vi "SMR_LabVIEW_V8.5.vi"() -> ()   [LabVIEW 2025]
uses:
  <vilib>/DAQmx/write.llb/DAQmx Write (Analog DBL 1Chan 1Samp).vi
  <vilib>/DAQmx/read.llb/DAQmx Read (Analog 1D DBL NChan 1Samp).vi
  <vilib>/DAQmx/read.llb/DAQmx Read (Analog 2D DBL NChan NSamp).vi
  <vilib>/Analysis/baseanly.llb/Mean (DBL).vi
  <vilib>/DAQmx/create/channels.llb/DAQmx Create Channel (AI-Temperature-Thermocouple).vi
  <vilib>/DAQmx/create/channels.llb/DAQmx Create Channel (AI-Voltage-Basic).vi
  <vilib>/DAQmx/create/channels.llb/DAQmx Create Channel (AO-Voltage-Basic).vi
  <vilib>/DAQmx/miscellaneous.llb/DAQmx Fill In Error Info.vi
  <vilib>/DAQmx/configure/timing.llb/DAQmx Timing (Sample Clock).vi
  <vilib>/addons/control/pid/pid.llb/PID (DBL).vi
  <vilib>/measure/maspectr.llb/FFT Power Spectrum and PSD for 1 Chan.vi
  <vilib>/measure/matone.llb/Extract Single Tone Information 1 Chan.vi
  <vilib>/addons/control/pid/NI_PID_pid.lvlib
  <vilib>/Analysis/NI_AALBase.lvlib
  <vilib>/ptbypt/NI_PtbyPt.lvlib
  <vilib>/measure/NI_MAPro.lvlib
panel:
  out "HW Valve Command (V)":dbl
  in  "HX Flow Setpoint (GPM)":dbl
  in  "Manual HW Valve Voltage (V)":dbl
  in  "HW Valve: Manual / PID":bool
  in  "PID gains for HW Valve":T1={"proportional gain (Kc)"=1.0, "integral time (Ti, min)"=0.01, "derivative time (Td, min)"=0.0} {"derivative time (Td, min)" format="%.3f"; "integral time (Ti, min)" format="%.3f"; "proportional gain (Kc)" format="%.3f"}
  out "Rod Power (W)":dbl
  out "Current Through Rod (A)":dbl
  out "Time in Steady State (s)":dbl
  in  "Steady-State Dwell (s)":dbl
  out "Main Loop Flow (GPM)":dbl
  out "FM Amplitude":dbl
  out "FM Frequency":dbl
  out "Spectrum":cluster{"f0":dbl, "df":dbl, "magnitude":dbl[]}(graph)
  out "Raw Signal":waveform(dbl)(graph)
  out "Smoothed HX Flow (GPM)":dbl
  out "Flow History":dbl(graph)
  out "HX Flow (GPM)":dbl
  out "Voltage Across Rod (V)":dbl format="%0.2f"
  out "Current Run Folder":path
  in  "Log Root Folder":path=path "C:/Users/LocalUser/Documents/GitHub/thermal-loop/resources/v0.1.1/data/001"
  out "Raw NI9201 \nVoltage Display":T2
  in  "Loop Period (ms)":dbl=1000.0
  in  "Stop":bool
  out "Auto Steady State Threshold (deg C/min)":dbl
  out "Max dT/dt (deg C/min)":dbl
  out "Temp Change Rate (deg C/min)":dbl
  out "5-Min Baseline Complete":bool
  out "Rate Window Ready":bool
  out "Steady State":bool
  in  "Voltage Limit (V)":dbl=10.0
  in  "Temperature Limit (C)":dbl=50.0
  in  "Pressure Limit (psi)":dbl=15.0
  out "Max Voltage":bool
  out "Max Temperature":bool
  out "Max Pressure":bool
  out "Heat Exchanger Pressure History":dbl(graph)
  out "Main Loop Pressure History":T3(graph)
  out "Overall Avg Pressure (psi)":dbl
  out "Heat Exchanger Pressure P6 (psi)":dbl
  out "Main Loop Avg Pressure (psi)":dbl
  out "Pressure Display":T4
  out "Overall Pressure History":T5(graph)
  out "Max Loop Pressure (psi)":dbl
  out "Heat Exchanger Temperature History":cluster{"Waveform":dbl, "Waveform":dbl}(graph)
  out "Main Loop Temeperature History":T6(graph)
  out "Heat Exchanger Avg Temp (deg C)":dbl
  out "Temperature Display":T7
  out "Overall Temperature History":T8(graph)
  out "Overall Avg Temp (deg C)":dbl
  out "Max Loop Temp (deg C)":dbl
  out "Final P-Valve Voltage (V)":dbl
  out "PID Trim Voltage (V)":dbl
  in  "PID Temp Setpoint (deg C)":dbl
  in  "Auto PID Enable":bool
  in  "Manual P-Valve Voltage (V)":dbl min=0.0 max=10.0
  out "Main Loop Avg Temp (deg C)":dbl
  # "HoneyWell Valve Control"
  # "Heat Exchanger Flow"
  # "Control/Troubleshoot"
  # "Steady State"
  # "Emergency Indicators"
  # "Pressure"
  # "Temperature"
  # "Proportional Valve Control"
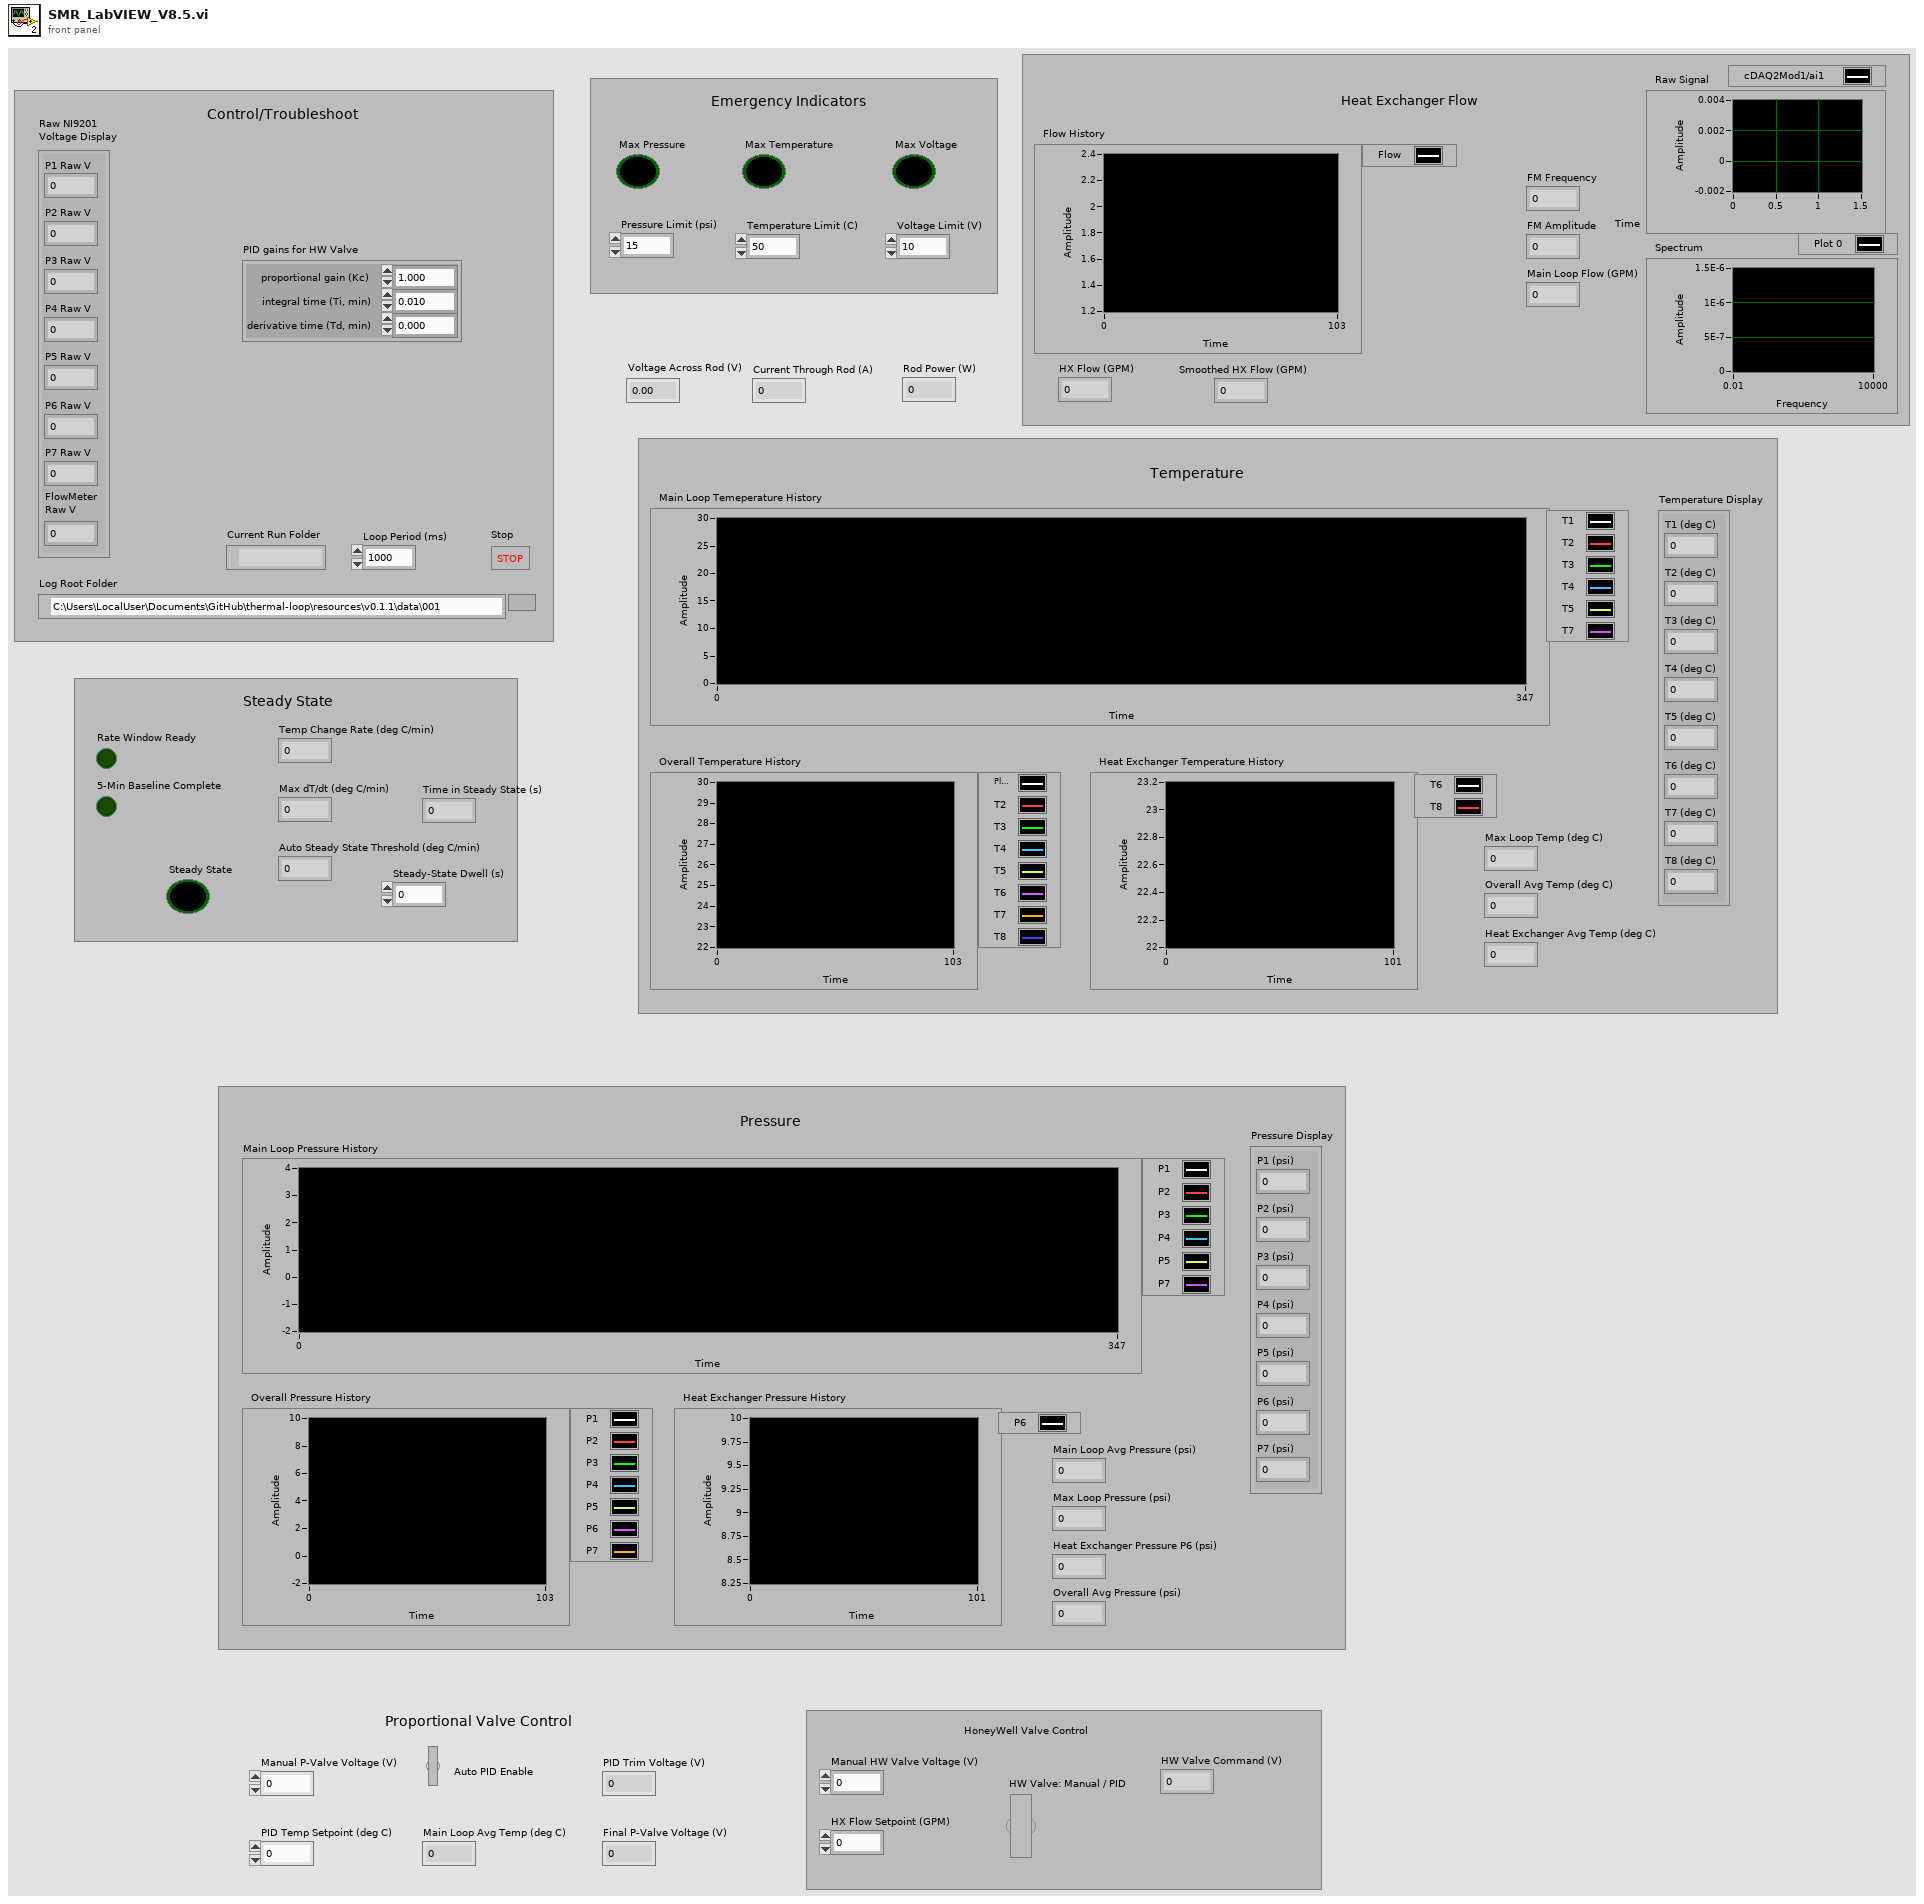
[diagram p1: front panel]
types:
  T1 = cluster{"proportional gain (Kc)":dbl, "integral time (Ti, min)":dbl, "derivative time (Td, min)":dbl}
  T2 = cluster{"P1 Raw V":dbl, "P2 Raw V":dbl, "P3 Raw V":dbl, "P4 Raw V":dbl, "P5 Raw V":dbl, "P6 Raw V":dbl, "P7 Raw V":dbl, "FlowMeter\nRaw V":dbl}
  T3 = cluster{"P1":dbl, "P2":dbl, "P3":dbl, "P4":dbl, "P5":dbl, "P7":dbl}
  T4 = cluster{"P1 (psi)":dbl, "P2 (psi)":dbl, "P3 (psi)":dbl, "P4 (psi)":dbl, "P5 (psi)":dbl, "P6 (psi)":dbl, "P7 (psi)":dbl}
  T5 = cluster{"P1":dbl, "P2":dbl, "P3":dbl, "P4":dbl, "P5":dbl, "P6":dbl, "P7":dbl}
  T6 = cluster{"Waveform":dbl, "Waveform":dbl, "Waveform":dbl, "Waveform":dbl, "Waveform":dbl, "Waveform":dbl}
  T7 = cluster{"T1 (deg C)":dbl, "T2 (deg C)":dbl, "T3 (deg C)":dbl, "T4 (deg C)":dbl, "T5 (deg C)":dbl, "T6 (deg C)":dbl, "T7 (deg C)":dbl, "T8 (deg C)":dbl}
  T8 = cluster{"Waveform":dbl, "Waveform":dbl, "Waveform":dbl, "Waveform":dbl, "Waveform":dbl, "Waveform":dbl, "Waveform":dbl, "Waveform":dbl}
  T9 = enum16{"open", "replace", "create", "open or create", "replace or create", "replace or create with confirmation"}
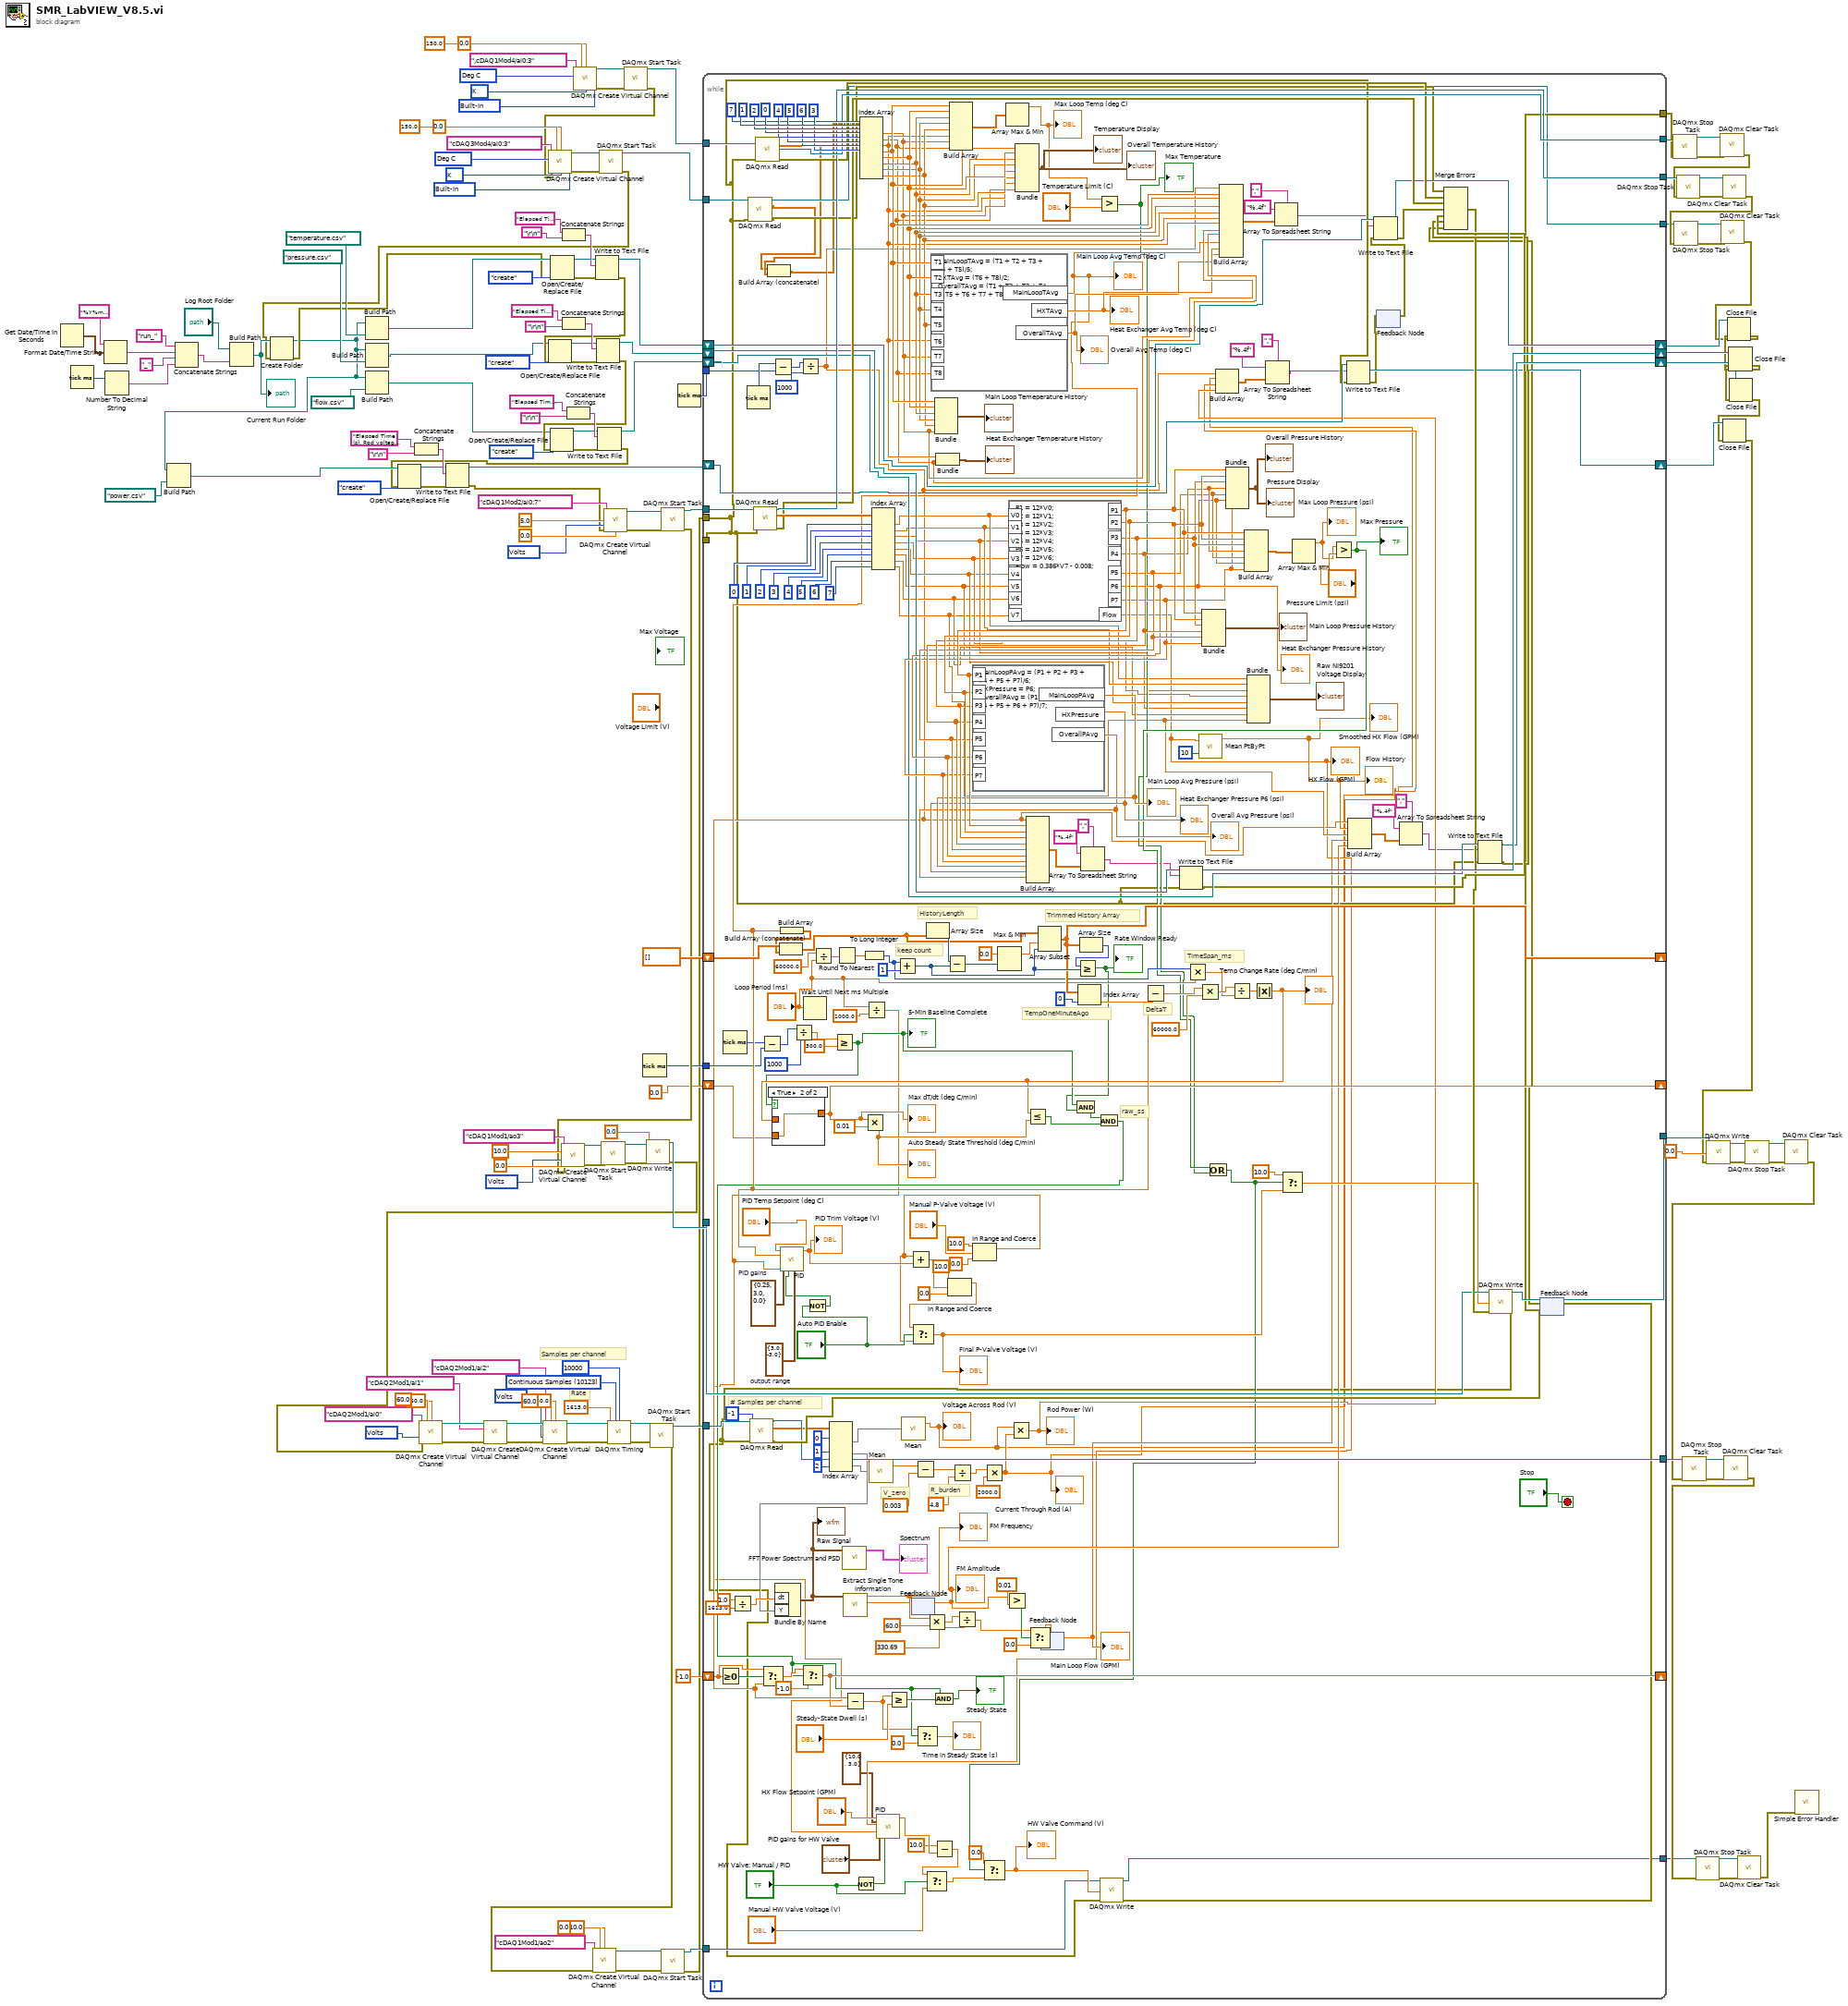
[diagram p0: block diagram]
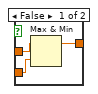
[diagram p2: hidden frame]
diagram:
  w17 = 10348 items=["Volts"=10348, "From Custom Scale"=10065] ("units")
  w34 = 10200 items=["Built-In"=10200, "Constant Value"=10116, "Channel"=10113] ("cjc source")
  w35 = 10073 items=["J"=10072, "K"=10073, "N"=10077, "R"=10082, "S"=10085, "T"=10086, "B"=10047, "E"=10055] ("thermocouple type")
  w36 = 10143 items=["Deg C"=10143, "Deg F"=10144, "Kelvins"=10325, "Deg R"=10145, "From Custom Scale"=10065] ("units")
  w66 = 10123 items=["Finite Samples"=10178, "Continuous Samples"=10123, "Hardware Timed Single Point"=12522] ("sample mode")
  w68 = 10348 items=["Volts"=10348, "From Custom Scale"=10065] ("units")
  w87 = 10348 items=["Volts"=10348, "From Custom Scale"=10065] ("units")
  w149 = 10200 items=["Built-In"=10200, "Constant Value"=10116, "Channel"=10113] ("cjc source")
  w150 = 10073 items=["J"=10072, "K"=10073, "N"=10077, "R"=10082, "S"=10085, "T"=10086, "B"=10047, "E"=10055] ("thermocouple type")
  w151 = 10143 items=["Deg C"=10143, "Deg F"=10144, "Kelvins"=10325, "Deg R"=10145, "From Custom Scale"=10065] ("units")
  w158 = 10348 items=["Volts"=10348, "From Custom Scale"=10065] ("units")
  # "Samples per channel"
  # "Rate"
  n1 = Get Date/Time In Seconds() -> (seconds since 1Jan1904=w108:timestamp)
  n2 = Tick Count (ms)() -> (millisecond timer value=w106:u32)
  n3 = Format Date/Time String(time format string (%c)="%Y%m%d_%H%M%S", seconds (now)=w108) -> (date/time string=w103:string)  [unwired: 1 in]
  n4 = Number To Decimal String(number=w106) -> (decimal integer string=w104:string)  [unwired: 1 in]
  n5 = Concatenate Strings("run_" ("string"), w103, "_" ("string"), w104) -> (w100:string)
  n6 = Build Path(base path="Log Root Folder", name or relative path=w100) -> (appended path=w99:path)
  "Current Run Folder" <- w99
  n7 = Concatenate Strings("Elapsed Time (s), Rod voltage (V), Rod Current (A), Rod Power (W)", "\r\n") -> (w53:string)
  n8 = Concatenate Strings("Elapsed Time (s),T1 (deg C),T2 (deg C),T3 (deg C),T4 (deg C),T5 (deg C),T6 (deg C),T7 (deg C),T8 (deg C),Main Loop Avg Temp (deg C),HX Avg Temp (deg C),Overall Avg Temp (deg C)", "\r\n") -> (w132:string)
  n9 = Concatenate Strings("Elapsed Time (s),P1 (psi),P2 (psi),P3 (psi),P4 (psi),P5 (psi),P6 (psi),P7 (psi),Main Loop Avg Pressure (psi),HX Pressure (psi),Overall Avg Pressure (psi)", "\r\n") -> (w130:string)
  n10 = Concatenate Strings("Elapsed Time (s),Heat Exchanger Flow (GPM),Flow Raw Voltage (V), Main Loop Flow (GPM), Flow Signal Amplitude (V)", "\r\n") -> (w126:string)
  n11 = call-poly <vilib>:"DAQmx Create Virtual Channel.vi"("maximum value"=150.0, "minimum value"=0.0, "physical channels"=tag ",cDAQ1Mod4/ai0:3", "cjc source"=w149, "units"=w151, "thermocouple type"=w150) -> ("task out"=w148:refnum<k21>, "error out"=w147:errorcluster)  [unwired: 8 in]
  n12 = call <vilib>:"DAQmx Start Task.vi"("task/channels in"=w148, "error in"=w147) -> ("task out"=w146:refnum<k21>, "error out"=w30:errorcluster)  [unwired: 12 in]
  n13 = call-poly <vilib>:"DAQmx Create Virtual Channel.vi"("maximum value"=150.0, "minimum value"=0.0, "physical channels"=tag "cDAQ3Mod4/ai0:3", "cjc source"=w34, "units"=w36, "error in"=w30, "thermocouple type"=w35) -> ("task out"=w33:refnum<k21>, "error out"=w32:errorcluster)  [unwired: 7 in]
  n14 = call <vilib>:"DAQmx Start Task.vi"("task/channels in"=w33, "error in"=w32) -> ("task out"=w28:refnum<k21>, "error out"=w29:errorcluster)  [unwired: 12 in]
  n15 = Create Folder(path (use dialog)=w99, error in=w29) -> (created path=w47:path, error out=w92:errorcluster)  [unwired: 1 in, 1 out]
  n16 = Build Path(base path=w47, name or relative path=path "power.csv") -> (appended path=w48:path)
  n17 = Build Path(base path=w47, name or relative path=path "temperature.csv") -> (appended path=w98:path)
  n18 = Build Path(base path=w47, name or relative path=path "pressure.csv") -> (appended path=w97:path)
  n19 = Build Path(base path=w47, name or relative path=path "flow.csv") -> (appended path=w96:path)
  n20 = Open/Create/Replace File(file path (use dialog)=w98, error in=w92, operation (0:open)=T9."create") -> (refnum out=w131:refnum<file>, error out=w115:errorcluster)  [unwired: 3 in, 1 out]
  n21 = Write to Text File(file (use dialog)=w131, text=w132, error in=w115) -> (refnum out=w122:refnum<file>, error out=w114:errorcluster)  [unwired: 1 in, 1 out]
  n22 = Open/Create/Replace File(file path (use dialog)=w97, error in=w114, operation (0:open)=T9."create") -> (refnum out=w129:refnum<file>, error out=w113:errorcluster)  [unwired: 3 in, 1 out]
  n23 = Write to Text File(file (use dialog)=w129, text=w130, error in=w113) -> (refnum out=w121:refnum<file>, error out=w112:errorcluster)  [unwired: 1 in, 1 out]
  n24 = Open/Create/Replace File(file path (use dialog)=w96, error in=w112, operation (0:open)=T9."create") -> (refnum out=w125:refnum<file>, error out=w111:errorcluster)  [unwired: 3 in, 1 out]
  n25 = Write to Text File(file (use dialog)=w125, text=w126, error in=w111) -> (refnum out=w120:refnum<file>, error out=w45:errorcluster)  [unwired: 1 in, 1 out]
  n26 = Open/Create/Replace File(file path (use dialog)=w48, error in=w45, operation (0:open)=T9."create") -> (refnum out=w52:refnum<file>, error out=w49:errorcluster)  [unwired: 3 in, 1 out]
  n27 = Write to Text File(file (use dialog)=w52, text=w53, error in=w49) -> (refnum out=w43:refnum<file>, error out=w44:errorcluster)  [unwired: 1 in, 1 out]
  n28 = call-poly <vilib>:"DAQmx Create Virtual Channel.vi"("maximum value"=5.0, "minimum value"=0.0, "physical channels"=tag "cDAQ1Mod2/ai0:7", "units"=w158, "error in"=w44) -> ("task out"=w157:refnum<k21>, "error out"=w156:errorcluster)  [unwired: 9 in]
  n29 = Tick Count (ms)() -> (millisecond timer value=w73:u32)
  n30 = call <vilib>:"DAQmx Start Task.vi"("task/channels in"=w157, "error in"=w156) -> ("task out"=w155:refnum<k21>, "error out"=w80:errorcluster)  [unwired: 12 in]
  n31 = call-poly <vilib>:"DAQmx Create Virtual Channel.vi"("maximum value"=10.0, "minimum value"=0.0, "physical channels"=tag "cDAQ1Mod1/ao3", "units"=w87, "error in"=w80) -> ("task out"=w86:refnum<k21>, "error out"=w85:errorcluster)  [unwired: 9 in]
  n32 = call <vilib>:"DAQmx Start Task.vi"("task/channels in"=w86, "error in"=w85) -> ("task out"=w84:refnum<k21>, "error out"=w83:errorcluster)  [unwired: 12 in]
  n33 = call-poly <vilib>:"DAQmx Write.vi"("task/channels in"=w84, "data"=0.0, "error in"=w83) -> ("task out"=w81:refnum<k21>, "error out"=w60:errorcluster)  [unwired: 10 in, 1 out]
  n34 = call-poly <vilib>:"DAQmx Create Virtual Channel.vi"("maximum value"=60.0, "minimum value"=-60.0, "physical channels"=tag "cDAQ2Mod1/ai0", "units"=w68, "error in"=w60) -> ("task out"=w57:refnum<k21>, "error out"=w56:errorcluster)  [unwired: 9 in]
  n35 = call-poly <vilib>:"DAQmx Create Virtual Channel.vi"("task in"=w57, "physical channels"=tag "cDAQ2Mod1/ai1", "error in"=w56) -> ("task out"=w21:refnum<k21>, "error out"=w19:errorcluster)  [unwired: 11 in]
  n36 = call-poly <vilib>:"DAQmx Create Virtual Channel.vi"("task in"=w21, "maximum value"=60.0, "minimum value"=-60.0, "physical channels"=tag "cDAQ2Mod1/ai2", "units"=w17, "error in"=w19) -> ("task out"=w20:refnum<k21>, "error out"=w18:errorcluster)  [unwired: 8 in]
  n37 = call-poly <vilib>:"DAQmx Timing.vi"("task/channels in"=w20, "sample mode"=w66, "samples per channel"=10000, "rate"=1613.0, "error in"=w18) -> ("task out"=w64:refnum<k21>, "error out"=w63:errorcluster)  [unwired: 9 in]
  n38 = call <vilib>:"DAQmx Start Task.vi"("task/channels in"=w64, "error in"=w63) -> ("task out"=w59:refnum<k21>, "error out"=w8:errorcluster)  [unwired: 12 in]
  n39 = call-poly <vilib>:"DAQmx Create Virtual Channel.vi"("maximum value"=10.0, "minimum value"=0.0, "physical channels"=tag "cDAQ1Mod1/ao2", "error in"=w8) -> ("task out"=w11:refnum<k21>, "error out"=w10:errorcluster)  [unwired: 10 in]
  n40 = call <vilib>:"DAQmx Start Task.vi"("task/channels in"=w11, "error in"=w10) -> ("task out"=w9:refnum<k21>, "error out"=w7:errorcluster)  [unwired: 12 in]
  n41 = Tick Count (ms)() -> (millisecond timer value=w119:u32)
  n42 = while {
    tunnel: w155 -> [w397]
    tunnel: w146 -> [w380]
    tunnel: [w371] -> w145
    tunnel: [w202] -> _
    tunnel: [w370] -> w144
    tunnel: [w258] -> w143
    shift-right: [w349] -> w118
    shift-left: w122 -> [w350]
    shift-right: [w334] -> w117
    shift-left: w121 -> [w335]
    shift-right: [w329] -> w116
    shift-left: w120 -> [w330]
    tunnel: w119 -> [w366]
    shift-right: [w308] -> _
    shift-left: dbl[] [] -> [w321]
    tunnel: w81 -> [w290]
    tunnel: w7 -> [w202]
    tunnel: [w296] -> w78
    tunnel: w73 -> [w279]
    shift-right: [w272] -> _
    shift-left: 0.0 -> [w274]
    tunnel: w59 -> [w257]
    tunnel: [w256] -> w58
    shift-right: [w219] -> w42
    shift-left: w43 -> [w220]
    shift-right: [w211] -> _
    shift-left: -1.0 -> [w215]
    tunnel: w28 -> [w203]
    tunnel: [w200] -> w24
    tunnel: w9 -> [w179]
    tunnel: [w175] -> w2
    stop <- "Stop" stop-if-true
    w294 = cluster{"output high":dbl, "output low":dbl} {"output high"=3.0, "output low"=-3.0}  # output range
    w295 = T1 {"proportional gain (Kc)"=0.25, "integral time (Ti, min)"=3.0, "derivative time (Td, min)"=0.0}  # PID gains
    # "R_burden"
    # "V_zero"
    # "raw_ss"
    # "# Samples per channel"
    # "TimeSpan_ms"
    # "DeltaT"
    # "TempOneMinuteAgo"
    # "Trimmed History Array"
    # "HistoryLength"
    # "keep count"
    n43 = Greater Or Equal To 0?(x=w215) -> (x >= 0?=w216:bool)
    n44 = Tick Count (ms)() -> (millisecond timer value=w280:u32)
    n45 = Divide(x=1.0, y=1613.0) -> (x/y=w230:dbl)
    n46 = Tick Count (ms)() -> (millisecond timer value=w367:u32)
    n47 = call-poly <vilib>:"DAQmx Read.vi"("task/channels in"=w203, "error in"=w202) -> ("task out"=w200:refnum<k21>, "data"=w197:dbl[], "error out"=w201:errorcluster)  [unwired: 11 in]
    n48 = call-poly <vilib>:"DAQmx Read.vi"("task/channels in"=w397, "error in"=w202) -> ("task out"=w370:refnum<k21>, "data"=w388:dbl[], "error out"=w368:errorcluster)  [unwired: 11 in]
    n49 = call-poly <vilib>:"DAQmx Read.vi"("task/channels in"=w380, "error in"=w202) -> ("task out"=w371:refnum<k21>, "data"=w198:dbl[], "error out"=w369:errorcluster)  [unwired: 11 in]
    n50 = Subtract(x=w280, y=w279) -> (x-y=w278:u32)
    n51 = Build Array (concatenate)(w197, w198) -> (w199:dbl[])
    n52 = Subtract(x=w367, y=w366) -> (x-y=w365:u32)
    n53 = Divide(x=w278, y=u32 1000) -> (x/y=w276:dbl)
    n54 = Divide(x=w365, y=u32 1000) -> (x/y=w212:dbl)
    n55 = Select(t=w215, s=w216, f=w212) -> (s? t:f=w214:dbl)
    n56 = Wait Until Next ms Multiple(millisecond multiple="Loop Period (ms)") -> ()  [unwired: 1 out]
    n57 = Not(x="Auto PID Enable") -> (.not. x?=w291:bool)
    n58 = Divide(x=60000.0, y="Loop Period (ms)") -> (x/y=w318:dbl)
    n59 = Greater Or Equal?(x=w276, y=300.0) -> (x >= y?=w269:bool)
    "5-Min Baseline Complete" <- w269
    n60 = Round To Nearest(number=w318) -> (nearest integer value=w317:dbl)
    n61 = Not(x="HW Valve: Manual / PID") -> (.not. x?=w189:bool)
    n62 = Index Array(array=w199, index #1=7 ("index"), index #2=1 ("index"), index #3=2 ("index"), index #4=0 ("index"), index #5=4 ("index"), index #6=5 ("index"), index #7=6 ("index"), index #8=3 ("index")) -> (element #1=w357:dbl, element #2=w356:dbl, element #3=w358:dbl, element #4=w363:dbl, element #5=w362:dbl, element #6=w361:dbl, element #7=w360:dbl, element #8=w359:dbl)
    n63 = To Long Integer(number=w317) -> (32bit integer=w305:i32)
    n64 = Divide(x="Loop Period (ms)", y=1000.0) -> (x/y=w174:dbl)
    n65 = Index Array(array=w388, index #1=0 ("index"), index #2=1 ("index"), index #3=2 ("index"), index #4=3 ("index"), index #5=4 ("index"), index #6=5 ("index"), index #7=6 ("index"), index #8=7 ("index")) -> (element #1=w255:dbl, element #2=w254:dbl, element #3=w253:dbl, element #4=w252:dbl, element #5=w251:dbl, element #6=w250:dbl, element #7=w249:dbl, element #8=w248:dbl)
    n66 = Add(x=w305, y=1) -> (x+y=w310:i32)
    n67 = feedback #1() -> (w226:dbl)  [unwired: 1 in]
    "FM Amplitude" <- w226
    n68 = formula code="MainLoopTAvg = (T1 + T2 + T3 + T4 + T5)/5;\nHXTAvg = (T6 + T8)/2;\nOverallTAvg = (T1 + T2 + T3 + T4 + T5 + T6 + T7 + T8)/8;"("T1"=w363, "T2"=w362, "T3"=w361, "T4"=w360, "T5"=w359, "T6"=w358, "T7"=w357, "T8"=w356) -> ("MainLoopTAvg"=w282:dbl, "HXTAvg"=w355:dbl, "OverallTAvg"=w354:dbl)
    "Overall Avg Temp (deg C)" <- w354
    "Main Loop Avg Temp (deg C)" <- w282
    "Heat Exchanger Avg Temp (deg C)" <- w355
    n69 = Build Array(w282) -> (w320:dbl[])
    n70 = Build Array (concatenate)(w321, w320) -> (w312:dbl[])
    n71 = call-poly <vilib>:"PID.vi"("reinitialize? (F)"=w291, "output range"=w294, "dt (s)"=w174, "PID gains"=w295, "process variable"=w282, "setpoint"="PID Temp Setpoint (deg C)") -> ("output"=w289:dbl)  [unwired: 4 in, 1 out]
    "PID Trim Voltage (V)" <- w289
    n72 = Array Size(array=w312) -> (size(s)=w315:i32)
    n73 = Bundle("Waveform"=w363, "Waveform"=w362, "Waveform"=w361, "Waveform"=w360, "Waveform"=w359, "Waveform"=w357) -> (→"Main Loop Temeperature History":T6)  [unwired: 1 in]
    n74 = Bundle("Waveform"=w358, "Waveform"=w356) -> (→"Heat Exchanger Temperature History":cluster{"Waveform":dbl, "Waveform":dbl})  [unwired: 1 in]
    n75 = Subtract(x=w315, y=w310) -> (x-y=w313:i32)
    n76 = Build Array(w363, w362, w361, w360, w359, w358, w357, w356) -> (w398:dbl[])
    n77 = In Range and Coerce(upper limit=10.0, x="Manual P-Valve Voltage (V)", lower limit=0.0) -> (coerced(x)=w284:dbl)  [unwired: 1 out]
    n78 = Add(x=w284, y=w289) -> (x+y=w288:dbl)
    n79 = In Range and Coerce(upper limit=10.0, x=w288, lower limit=0.0) -> (coerced(x)=w283:dbl)  [unwired: 1 out]
    n80 = Select(t=w283, s="Auto PID Enable", f=w284) -> (s? t:f=w261:dbl)
    "Final P-Valve Voltage (V)" <- w261
    n81 = Max & Min(x=0.0, y=w313) -> (max(x,y)=w311:dbl)  [unwired: 1 out]
    n82 = Array Max & Min(array=w398) -> (max value=w323:dbl)  [unwired: 3 out]
    "Max Loop Temp (deg C)" <- w323
    n83 = Greater?(x=w226, y=0.01) -> (0:w234:bool)
    n84 = formula code="P1 = 12*V0;\nP2 = 12*V1;\nP3 = 12*V2;\nP4 = 12*V3;\nP5 = 12*V4;\nP6 = 12*V5; \nP7 = 12*V6;\nFlow = 0.386*V7 - 0.008;"("V0"=w255, "V1"=w254, "V2"=w253, "V3"=w252, "V4"=w251, "V5"=w250, "V6"=w249, "V7"=w248) -> ("P1"=w348:dbl, "P2"=w347:dbl, "P3"=w346:dbl, "P4"=w345:dbl, "P5"=w344:dbl, "P6"=w343:dbl, "P7"=w342:dbl, "Flow"=w192:dbl)
    "HX Flow (GPM)" <- w192
    "Heat Exchanger Pressure History" <- w343
    n85 = call-poly <vilib>:"PID.vi"("reinitialize? (F)"=w189, "output range"=cluster{"output high":dbl, "output low":dbl} {"output high"=10.0, "output low"=3.0}, "dt (s)"=w174, "PID gains"="PID gains for HW Valve", "process variable"=w192, "setpoint"="HX Flow Setpoint (GPM)") -> ("output"=w188:dbl)  [unwired: 4 in, 1 out]
    n86 = Subtract(x=10.0, y=w188) -> (x-y=w185:dbl)
    n87 = Select(t=w185, s="HW Valve: Manual / PID", f="Manual HW Valve Voltage (V)") -> (s? t:f=w182:dbl)
    n88 = formula code="MainLoopPAvg = (P1 + P2 + P3 + P4 + P5 + P7)/6;\nHXPressure = P6;\nOverallPAvg = (P1 + P2 + P3 + P4 + P5 + P6 + P7)/7;"("P1"=w348, "P2"=w347, "P3"=w346, "P4"=w345, "P5"=w344, "P6"=w343, "P7"=w342) -> ("MainLoopPAvg"=w341:dbl, "HXPressure"=w340:dbl, "OverallPAvg"=w339:dbl)
    "Overall Avg Pressure (psi)" <- w339
    "Heat Exchanger Pressure P6 (psi)" <- w340
    "Main Loop Avg Pressure (psi)" <- w341
    n89 = Bundle("Waveform"=w363, "Waveform"=w362, "Waveform"=w361, "Waveform"=w360, "Waveform"=w359, "Waveform"=w358, "Waveform"=w357, "Waveform"=w356) -> (→"Overall Temperature History" →"Temperature Display":T8)  [unwired: 1 in]
    n90 = Build Array(w212, w348, w347, w346, w345, w344, w343, w342, w341, w340, w339) -> (w338:dbl[])
    n91 = Array Subset(array=w312, index=w311, length=w310) -> (w308:dbl[])
    n92 = feedback #2() -> (w224:dbl)  [unwired: 1 in]
    "Main Loop Flow (GPM)" <- w224
    n93 = Index Array(array=w308, index=0) -> (element=w306:dbl)
    n94 = Array Size(array=w308) -> (size(s)=w309:i32)
    n95 = Greater Or Equal?(x=w309, y=w310) -> (x >= y?=w268:bool)
    "Rate Window Ready" <- w268
    n96 = And(x=w269, y=w268) -> (x .and. y?=w267:bool)
    n97 = Array To Spreadsheet String(delimiter (Tab)=",", array=w338, 3:"%.4f" ("format string")) -> (spreadsheet string=w170:string)
    n98 = Greater?(x=w323, y="Temperature Limit (C)") -> (0:w264:bool)
    "Max Temperature" <- w264
    n99 = Subtract(x=w282, y=w306) -> (x-y=w304:dbl)
    n100 = Write to Text File(file (use dialog)=w335, text=w170, error in=w202) -> (refnum out=w334:refnum<file>, error out=w327:errorcluster)  [unwired: 1 in, 1 out]
    n101 = Multiply(x=w305, y="Loop Period (ms)") -> (x*y=w301:dbl)
    n102 = Multiply(x=w304, y=60000.0) -> (x*y=w302:dbl)
    n103 = call <vilib>:"Mean PtByPt.vi"("x"=w192, "sample length"=10) -> ("mean"=w246:dbl)  [unwired: 2 in, 1 out]
    "Flow History" <- w246
    "Smoothed HX Flow (GPM)" <- w246
    n104 = Bundle("P1"=w348, "P2"=w347, "P3"=w346, "P4"=w345, "P5"=w344, "P7"=w342) -> (→"Main Loop Pressure History":T3)  [unwired: 1 in]
    n105 = Build Array(w212, w363, w362, w361, w360, w359, w358, w357, w356, w282, w355, w354) -> (w353:dbl[])
    n106 = Bundle("P1"=w348, "P2"=w347, "P3"=w346, "P4"=w345, "P5"=w344, "P6"=w343, "P7"=w342) -> (→"Overall Pressure History" →"Pressure Display":T5)  [unwired: 1 in]
    n107 = Divide(x=w302, y=w301) -> (x/y=w300:dbl)
    n108 = Build Array(w348, w347, w346, w345, w344, w343, w342) -> (w387:dbl[])
    n109 = Bundle("Waveform"=w255, "Waveform"=w254, "Waveform"=w253, "Waveform"=w252, "Waveform"=w251, "Waveform"=w250, "Waveform"=w249, "Waveform"=w248) -> (→"Raw NI9201 \nVoltage Display":T8)  [unwired: 1 in]
    n110 = Absolute Value(x=w300) -> (abs(x)=w271:dbl)
    "Temp Change Rate (deg C/min)" <- w271
    n111 = case shown="True" w269 {
      tunnel: w274 -> [w402 w403]
      tunnel: w271 -> [w401 _]
      tunnel: [w400 w403] -> w272
      frame False {
        n112 = Max & Min(x=w401, y=w402) -> (max(x,y)=w400:dbl)  [unwired: 1 out]
      }
      frame True {
      }
    }
    "Max dT/dt (deg C/min)" <- w272
    n113 = Multiply(x=w272, y=0.01) -> (x*y=w270:dbl)
    "Auto Steady State Threshold (deg C/min)" <- w270
    n114 = Less Or Equal?(x=w271, y=w270) -> (x <= y?=w266:bool)
    n115 = And(x=w267, y=w266) -> (x .and. y?=w207:bool)
    n116 = Select(t=w214, s=w207, f=-1.0) -> (s? t:f=w211:dbl)
    n117 = Subtract(x=w212, y=w211) -> (x-y=w206:dbl)
    n118 = Greater Or Equal?(x=w206, y="Steady-State Dwell (s)") -> (x >= y?=w209:bool)
    n119 = Select(t=w206, s=w207, f=0.0) -> (s? t:f=→"Time in Steady State (s)":dbl)
    n120 = And(x=w207, y=w209) -> (x .and. y?=→"Steady State":bool)
    n121 = Array To Spreadsheet String(delimiter (Tab)=",", array=w353, 3:"%.4f" ("format string")) -> (spreadsheet string=w171:string)
    n122 = Array Max & Min(array=w387) -> (max value=w324:dbl)  [unwired: 3 out]
    "Max Loop Pressure (psi)" <- w324
    n123 = Greater?(x=w324, y="Pressure Limit (psi)") -> (0:w265:bool)
    "Max Pressure" <- w265
    n124 = Or(x=w265, y=w264) -> (x .or. y?=w183:bool)
    n125 = Select(t=0.0, s=w183, f=w182) -> (s? t:f=w180:dbl)
    "HW Valve Command (V)" <- w180
    n126 = Select(t=10.0, s=w183, f=w261) -> (s? t:f=w260:dbl)
    n127 = Build Array(w212, w246, w248, w224, w226) -> (w333:dbl[])
    n128 = feedback #3() -> (w217:errorcluster)  [unwired: 1 in]
    n129 = Write to Text File(file (use dialog)=w350, text=w171, error in=w217) -> (refnum out=w349:refnum<file>, error out=w328:errorcluster)  [unwired: 1 in, 1 out]
    n130 = Array To Spreadsheet String(delimiter (Tab)=",", array=w333, 3:"%.4f" ("format string")) -> (spreadsheet string=w173:string)
    n131 = Write to Text File(file (use dialog)=w330, text=w173, error in=w202) -> (refnum out=w329:refnum<file>, error out=w326:errorcluster)  [unwired: 1 in, 1 out]
    n132 = feedback #4() -> (w176:errorcluster)  [unwired: 1 in]
    n133 = Merge Errors(w201, w369, w368, w328, w327, w326, w176) -> (w297:errorcluster)
    n134 = call-poly <vilib>:"DAQmx Write.vi"("task/channels in"=w290, "data"=w260, "error in"=w297) -> ("task out"=w296:refnum<k21>, "error out"=w178:errorcluster)  [unwired: 10 in, 1 out]
    n135 = call-poly <vilib>:"DAQmx Read.vi"("task/channels in"=w257, "number of samples per channel"=-1, "error in"=w178) -> ("task out"=w256:refnum<k21>, "data"=w245:dbl[][], "error out"=w258:errorcluster)  [unwired: 10 in]
    n136 = Index Array(array=w245, index (row) #1=0 ("index (row)"), index (row) #2=1 ("index (row)"), index (row) #3=2 ("index (row)")) -> (element #1=w244:dbl[], element #2=w229:dbl[], element #3=w195:dbl[])  [unwired: 3 in]
    n137 = Bundle By Name("dt"=w230, "Y"=w229) -> (w228:waveform(dbl))  [unwired: 1 in]
    "Raw Signal" <- w228
    n138 = call-poly <vilib>:"FFT Power Spectrum and PSD.vi"("time signal"=w228) -> ("Power Spectrum / PSD"=→"Spectrum":cluster{"f0":dbl, "df":dbl, "magnitude":dbl[]})  [unwired: 7 in, 3 out]
    n139 = call-poly <vilib>:"Extract Single Tone Information.vi"("time signal in"=w228) -> ("detected amplitude"=w227:dbl, "detected frequency"=w240:dbl)  [unwired: 5 in, 4 out]
    "FM Frequency" <- w240
    n140 = call-poly <vilib>:"Mean.vi"("X"=w195) -> ("mean"=w169:dbl)  [unwired: 1 out]
    n141 = call-poly <vilib>:"Mean.vi"("X"=w244) -> ("mean"=w162:dbl)  [unwired: 1 out]
    "Voltage Across Rod (V)" <- w162
    n142 = feedback-in #1(w227) -> ()
    n143 = Subtract(x=w169, y=0.003) -> (x-y=w167:dbl)
    n144 = Multiply(x=w240, y=60.0) -> (x*y=w238:dbl)
    n145 = Divide(x=w167, y=4.8) -> (x/y=w165:dbl)
    n146 = Divide(x=w238, y=330.69) -> (x/y=w233:dbl)
    n147 = Multiply(x=w165, y=2000.0) -> (x*y=w163:dbl)
    "Current Through Rod (A)" <- w163
    n148 = Multiply(x=w162, y=w163) -> (x*y=w194:dbl)
    "Rod Power (W)" <- w194
    n149 = Select(t=w233, s=w234, f=0.0) -> (s? t:f=w225:dbl)
    n150 = feedback-in #2(w225) -> ()
    n151 = call-poly <vilib>:"DAQmx Write.vi"("task/channels in"=w179, "data"=w180, "error in"=w178) -> ("task out"=w175:refnum<k21>, "error out"=w177:errorcluster)  [unwired: 10 in, 1 out]
    n152 = Build Array(w212, w162, w163, w194) -> (w221:dbl[])
    n153 = Array To Spreadsheet String(delimiter (Tab)=",", array=w221, 3:"%.4f" ("format string")) -> (spreadsheet string=w172:string)
    n154 = Write to Text File(file (use dialog)=w220, text=w172, error in=w202) -> (refnum out=w219:refnum<file>, error out=w218:errorcluster)  [unwired: 1 in, 1 out]
    n155 = feedback-in #3(w218) -> ()
    n156 = feedback-in #4(w177) -> ()
  }
  n157 = call <vilib>:"DAQmx Stop Task.vi"("task/channels in"=w145, "error in"=w143) -> ("task out"=w142:refnum<k21>, "error out"=w140:errorcluster)  [unwired: 12 in]
  n158 = call <vilib>:"DAQmx Clear Task.vi"("task in"=w142, "error in"=w140) -> ("error out"=w139:errorcluster)  [unwired: 13 in]
  n159 = call <vilib>:"DAQmx Stop Task.vi"("task/channels in"=w144, "error in"=w139) -> ("task out"=w141:refnum<k21>, "error out"=w138:errorcluster)  [unwired: 12 in]
  n160 = call <vilib>:"DAQmx Clear Task.vi"("task in"=w141, "error in"=w138) -> ("error out"=w27:errorcluster)  [unwired: 13 in]
  n161 = call <vilib>:"DAQmx Stop Task.vi"("task/channels in"=w24, "error in"=w27) -> ("task out"=w23:refnum<k21>, "error out"=w26:errorcluster)  [unwired: 12 in]
  n162 = call <vilib>:"DAQmx Clear Task.vi"("task in"=w23, "error in"=w26) -> ("error out"=w25:errorcluster)  [unwired: 13 in]
  n163 = Close File(refnum=w118, error in=w25) -> (error out=w110:errorcluster)  [unwired: 1 out]
  n164 = Close File(refnum=w117, error in=w110) -> (error out=w109:errorcluster)  [unwired: 1 out]
  n165 = Close File(refnum=w116, error in=w109) -> (error out=w41:errorcluster)  [unwired: 1 out]
  n166 = Close File(refnum=w42, error in=w41) -> (error out=w40:errorcluster)  [unwired: 1 out]
  n167 = call-poly <vilib>:"DAQmx Write.vi"("task/channels in"=w78, "data"=0.0, "error in"=w40) -> ("task out"=w77:refnum<k21>, "error out"=w75:errorcluster)  [unwired: 10 in, 1 out]
  n168 = call <vilib>:"DAQmx Stop Task.vi"("task/channels in"=w77, "error in"=w75) -> ("task out"=w76:refnum<k21>, "error out"=w74:errorcluster)  [unwired: 12 in]
  n169 = call <vilib>:"DAQmx Clear Task.vi"("task in"=w76, "error in"=w74) -> ("error out"=w6:errorcluster)  [unwired: 13 in]
  n170 = call <vilib>:"DAQmx Stop Task.vi"("task/channels in"=w58, "error in"=w6) -> ("task out"=w62:refnum<k21>, "error out"=w61:errorcluster)  [unwired: 12 in]
  n171 = call <vilib>:"DAQmx Clear Task.vi"("task in"=w62, "error in"=w61) -> ("error out"=w3:errorcluster)  [unwired: 13 in]
  n172 = call <vilib>:"DAQmx Stop Task.vi"("task/channels in"=w2, "error in"=w3) -> ("task out"=w5:refnum<k21>, "error out"=w4:errorcluster)  [unwired: 12 in]
  n173 = call <vilib>:"DAQmx Clear Task.vi"("task in"=w5, "error in"=w4) -> ("error out"=w1:errorcluster)  [unwired: 13 in]
  n174 = call <vilib>:"Simple Error Handler.vi"("error in (no error)"=w1) -> ()  [unwired: 4 in, 5 out]
